vi "OwnCompat20261012_Own20261012_GetObjectIdentity.vi"() -> ()   [LabVIEW 2024]
panel:
  out "error out":errorcluster caption="错误输出"
  out "vi_path":path
  out "uid":i32
  in  "object_id":u32
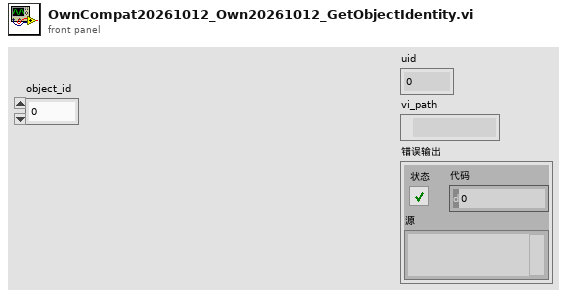
[diagram p1: front panel]
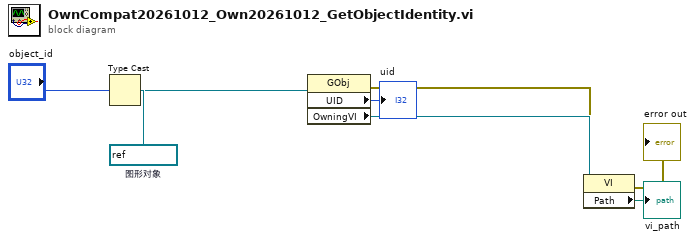
[diagram p0: block diagram]
diagram:
  w7 = refnum<vi> refnum  # 图形对象
  n1 = Type Cast ("强制类型转换")(type=w7, x="object_id") -> (*(type *) &x=w1:refnum<vi>)
  n2 = property on="属性节点" class="GObj"(reference=w1) -> (error out=w5:errorcluster, "UID"=→"uid":i32, "OwningVI"=w6:refnum<vi>)  [unwired: 1 in, 1 out]
  n3 = property class="VI"(reference=w6, error in=w5) -> (error out=→"error out":errorcluster, "Path"=→"vi_path":path)  [unwired: 1 out]
